vi "Test MQTT-3.2.2-2.vi"(8 "error in (no error)":errorcluster, 11 "Connection Config":refnum<class "Connection.lvclass">) -> (0 "error out":errorcluster, 3 "Connection Config dup":refnum<class "Connection.lvclass">)   [LabVIEW 2013]
uses:
  <vilib>/LabVIEW Open Source Project/MQTT Control Packets/Control Packets/CONNECT/CONNECT.lvclass
  <vilib>/LabVIEW Open Source Project/MQTT Control Packets/Control Packets/ControlPacket/ControlPacket.lvclass
  <vilib>/addons/_JKI Toolkits/Caraya/classes/Test/Test.lvclass
  <vilib>/LabVIEW Open Source Project/MQTT Control Packets/Control Packets/DISCONNECT/DISCONNECT.lvclass
  <vilib>/LabVIEW Open Source Project/MQTT Control Packets/Control Packets/CONNECT/ConnectFlags -- cluster.ctl
  <vilib>/LabVIEW Open Source Project/Connection/Connection/Connection.lvclass
  <vilib>/LabVIEW Open Source Project/MQTT Control Packets/Control Packets/CONNACK/CONNACK.lvclass
  <vilib>/addons/_JKI Toolkits/Caraya/classes/Assert/Assert.lvclass
  <vilib>/addons/_JKI Toolkits/Caraya/classes/Assert/Assert True.vi
  <vilib>/LabVIEW Open Source Project/MQTT Connection/MQTT_Connection/Connection/Connection.lvclass
panel:
  out "Bytes 2":u8[](array[numeric]) format="%08b"
  out "Bytes":u8[](array[numeric]) format="%08b"
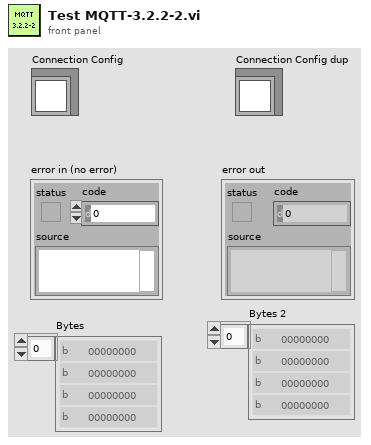
[diagram p1: front panel]
types:
  T1 = typedef "MQTT_Control_Packets.lvlib/CONNECT.lvclass/ConnectFlags -- cluster.ctl" = cluster{"Reserved":bool, "Clean Session":bool, "Will Flag":bool, "Will QoS 1":bool, "Will QoS 2":bool, "Will Retain":bool, "Password Flag":bool, "User Name Flag":bool}
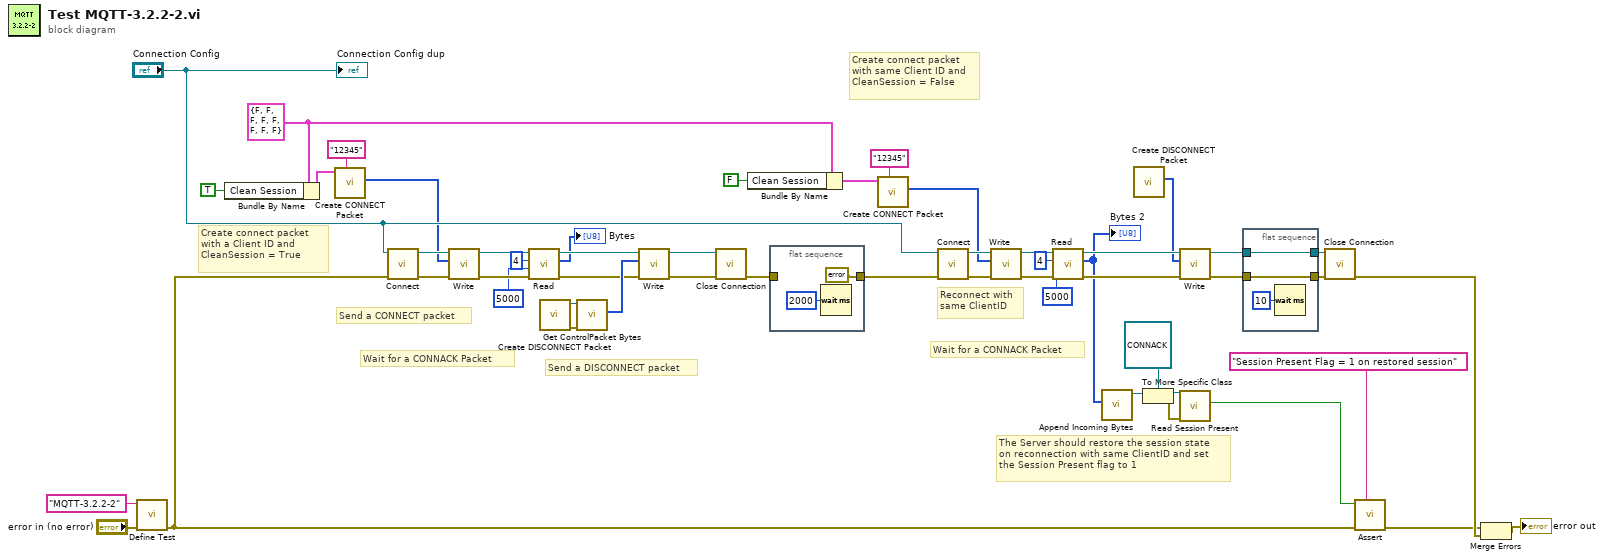
[diagram p0: block diagram]
diagram:
  w4 = T1 {"Reserved"=FALSE, "Clean Session"=FALSE, "Will Flag"=FALSE, "Will QoS 1"=FALSE, "Will QoS 2"=FALSE, "Will Retain"=FALSE, "Password Flag"=FALSE, "User Name Flag"=FALSE} ("Connect Flags")
  # "Create connect packet with same Client ID and CleanSession = False"
  # "Wait for a CONNACK Packet"
  # "The Server should restore the session state\non reconnection with same ClientID and set\nthe Session Present flag to 1"
  # "Reconnect with\nsame ClientID"
  # "Send a DISCONNECT packet"
  # "Wait for a CONNACK Packet"
  # "Create connect packet with a Client ID and CleanSession = True"
  # "Send a CONNECT packet"
  n1 = call <vilib>:"Define Test.vi"("error in (no error)"="error in (no error)", "Label (VI Title)"="MQTT-3.2.2-2") -> ("error out"=w9:errorcluster)  [unwired: 9 in]
  n2 = Bundle By Name(cluster=w4, "Clean Session"=TRUE) -> (w42:T1)
  n3 = call <vilib>:"Create CONNECT Packet.vi"("Client ID (empty: generate new)"="12345", "Connect Flags"=w42) -> ("Bytes Stream"=w2:u8[])  [unwired: 7 in, 2 out]
  n4 = call <vilib>:"Connect.vi"("error in (no error)"=w9, "Connection in"="Connection Config") -> ("error out"=w40:errorcluster, "Connection out"=w39:refnum<class "Connection.lvclass">)  [unwired: 8 in]
  n5 = call <vilib>:"Write.vi"("error in (no error)"=w40, "Bytes"=w2, "Connection in"=w39) -> ("error out"=w44:errorcluster, "Connection"=w45:refnum<class "Connection.lvclass">)  [unwired: 7 in]
  n6 = call <vilib>:"Read.vi"("error in (no error)"=w44, "timeout (2000 ms)"=5000 ("timeout (1000 ms)"), "bytes to read (100)"=4 ("bytes to read"), "TCPConnection in"=w45) -> ("error out"=w32:errorcluster, "Bytes"=→"Bytes":u8[], "TCPConnection out"=w33:refnum<class "Connection.lvclass">)  [unwired: 3 in, 2 out]
  n7 = call <vilib>:"Create DISCONNECT Packet.vi"() -> ("error out"=w49:errorcluster, "DISCONNECT"=w48:refnum<class "DISCONNECT.lvclass">)  [unwired: 9 in, 1 out]
  n8 = call <vilib>:"Get ControlPacket Bytes.vi"("error in (no error)"=w49, "ControlPacket"=w48) -> ("Bytes Stream"=w47:u8[])  [unwired: 6 in, 3 out]
  n9 = call <vilib>:"Write.vi"("error in (no error)"=w32, "Bytes"=w47, "Connection in"=w33) -> ("error out"=w22:errorcluster, "Connection"=w23:refnum<class "Connection.lvclass">)  [unwired: 7 in]
  n10 = call <vilib>:"Close Connection.vi"("error in (no error)"=w22, "Connection in"=w23) -> ("error out"=w21:errorcluster)  [unwired: 8 in, 1 out]
  n11 = Bundle By Name(cluster=w4, "Clean Session"=FALSE) -> (w3:T1)
  n12 = flat-sequence {
    tunnel: [errorcluster {"status"=FALSE, "code"=0, "source"=""} ("error out")] -> w20
    tunnel: w21 -> [_]
    frame #0 {
      n13 = Wait (ms)(milliseconds to wait=u32 2000) -> ()  [unwired: 1 out]
    }
  }
  n14 = call <vilib>:"Create CONNECT Packet.vi"("Client ID (empty: generate new)"="12345", "Connect Flags"=w3) -> ("Bytes Stream"=w1:u8[])  [unwired: 7 in, 2 out]
  n15 = call <vilib>:"Connect.vi"("error in (no error)"=w20, "Connection in"="Connection Config") -> ("error out"=w38:errorcluster, "Connection out"=w37:refnum<class "Connection.lvclass">)  [unwired: 8 in]
  n16 = call <vilib>:"Write.vi"("error in (no error)"=w38, "Bytes"=w1, "Connection in"=w37) -> ("error out"=w34:errorcluster, "Connection"=w35:refnum<class "Connection.lvclass">)  [unwired: 7 in]
  n17 = call <vilib>:"Read.vi"("error in (no error)"=w34, "timeout (2000 ms)"=5000 ("timeout (1000 ms)"), "bytes to read (100)"=4 ("bytes to read"), "TCPConnection in"=w35) -> ("error out"=w31:errorcluster, "Bytes"=w15:u8[], "TCPConnection out"=w30:refnum<class "Connection.lvclass">)  [unwired: 3 in, 2 out]
  "Bytes 2" <- w15
  n18 = call <vilib>:"Append Incoming Bytes.vi"("Incoming Packets"=w15) -> ("ControlPacket"=w13:refnum<class "ControlPacket.lvclass">)  [unwired: 7 in, 3 out]
  n19 = call <vilib>:"Create DISCONNECT Packet.vi"() -> ("Bytes Stream"=w16:u8[])  [unwired: 9 in, 2 out]
  n20 = To More Specific Class(target class=refnum<class "CONNACK.lvclass"> refnum ("CONNACK in"), reference=w13) -> (specific class reference=w11:refnum<class "CONNACK.lvclass">, error out=w14:errorcluster)  [unwired: 1 in]
  n21 = call <vilib>:"Write.vi"("error in (no error)"=w31, "Bytes"=w16, "Connection in"=w30) -> ("error out"=w27:errorcluster, "Connection"=w26:refnum<class "Connection.lvclass">)  [unwired: 7 in]
  n22 = call <vilib>:"Read Session Present.vi"("error in (no error)"=w14, "CONNACK in"=w11) -> ("Session Present"=w10:bool)  [unwired: 7 in, 2 out]
  n23 = flat-sequence {
    tunnel: w26 -> [w57]
    tunnel: [w57] -> w28
    tunnel: [w55] -> w29
    tunnel: w27 -> [w55]
    frame #0 {
      n24 = Wait (ms)(milliseconds to wait=u32 10) -> ()  [unwired: 1 out]
    }
  }
  n25 = call <vilib>:"Close Connection.vi"("error in (no error)"=w29, "Connection in"=w28) -> ("error out"=w25:errorcluster)  [unwired: 8 in, 1 out]
  n26 = call-poly <vilib>:"Assert.vi"("Label"="Session Present Flag = 1 on restored session", "error in (no error)"=w9, "True?"=w10) -> ("error out"=w8:errorcluster)  [unwired: 8 in]
  n27 = Merge Errors(w8, w25) -> (→"error out":errorcluster)
  "Connection Config dup" <- "Connection Config"
